vi "AssertLessThan_Tests.vi"(11 "error in":errorcluster) -> (15 "error out":errorcluster)   [LabVIEW 2016, in "DronaTest.lvlib"]
uses:
  DronaTest.lvlib
  APIs/Assert/AssertControlValue/LessOrEqual.vi
  <vilib>/addons/_JKI Toolkits/Caraya/classes/Assert/Assert Less Or Equal_Variant.vi
  APIs/Assert/AssertControlValue/Less.vi
  <vilib>/addons/_JKI Toolkits/Caraya/classes/Assert/Assert Less_Variant.vi
  <vilib>/addons/_JKI Toolkits/Caraya/classes/Assert/Assert Error.vi
  <vilib>/addons/_JKI Toolkits/Caraya/classes/Test/Test.lvclass
  Drona.lvlib
  <vilib>/addons/_JKI Toolkits/Caraya/classes/Assert/Assert.lvclass
  APIs/Assert/AssertControlValue/AssertControlValue.lvlib
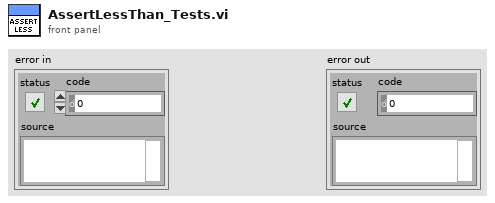
[diagram p1: front panel]
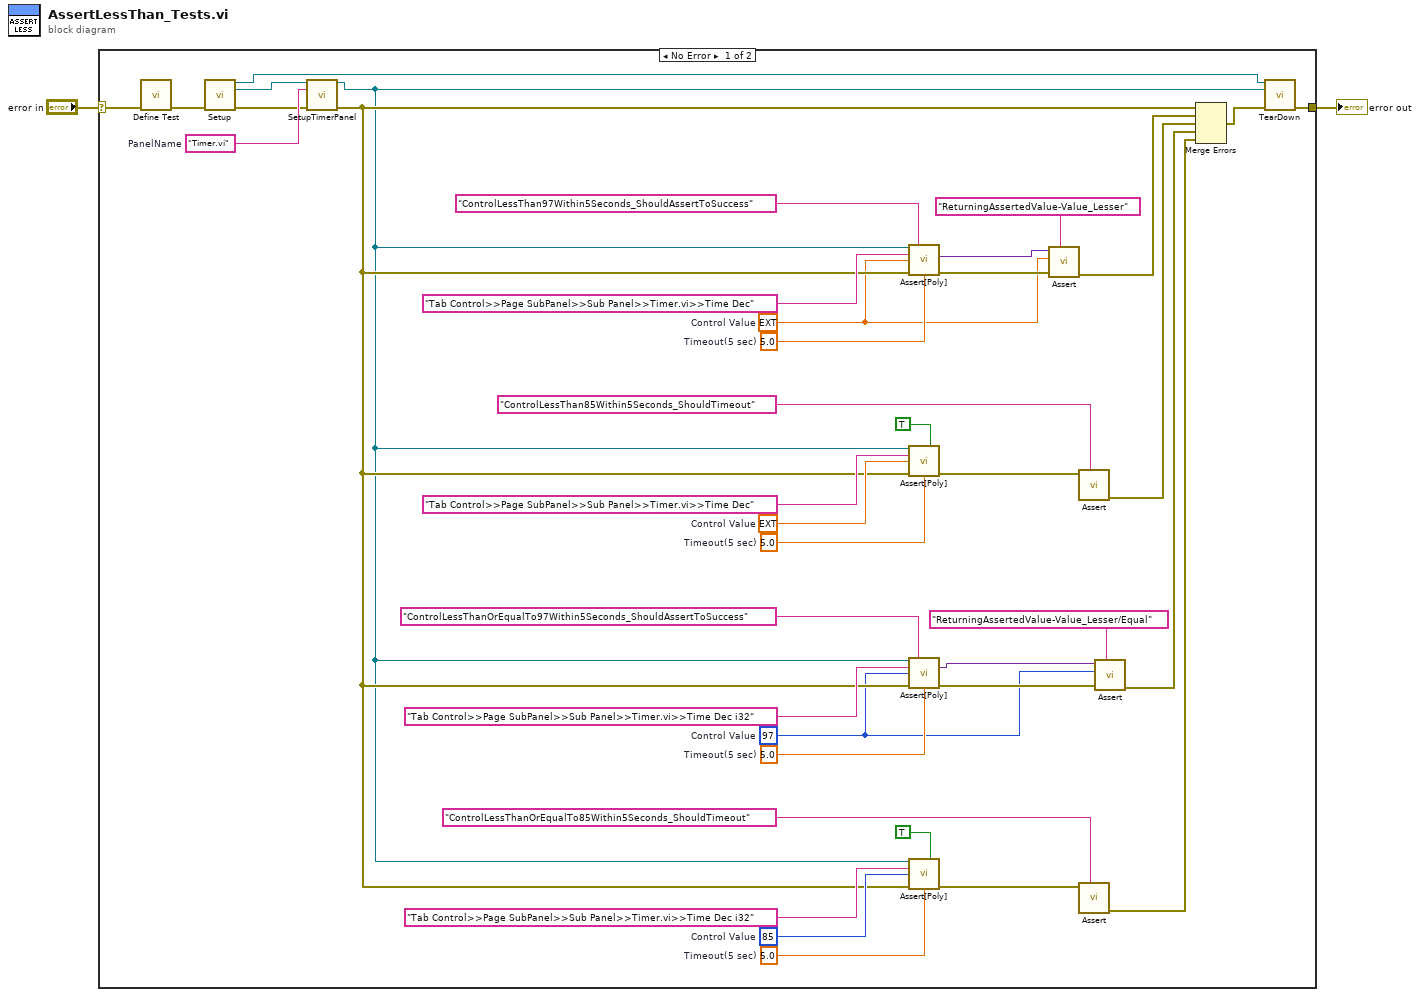
[diagram p0: block diagram]
diagram:
  n1 = case shown="No Error" "error in" {
    selector: "error in" -> [w42 w43]
    tunnel: [w17 w43] -> w1
    frame No Error {
      w21 = "Timer.vi"  # PanelName
      w35 = 5.0  # Timeout(5 sec)
      w3 = 97  # Control Value
      w36 = 5.0  # Timeout(5 sec)
      w37 = 85  # Control Value
      w30 = 5.0  # Timeout(5 sec)
      w9 = ext 97.0  # Control Value
      w29 = 5.0  # Timeout(5 sec)
      w28 = ext 85.0  # Control Value
      n2 = call <vilib>:"Define Test.vi"("error in (no error)"=w42) -> ("error out"=w16:errorcluster)  [unwired: 9 in, 1 out]
      n3 = call "Setup.vi"("error in (no error)"=w16) -> ("Application Ref"=w15:refnum<vi>, "VI out"=w19:refnum<vi>, "error out"=w20:errorcluster)  [unwired: 12 in]
      n4 = call "SetupTimerPanel.vi"("VI in"=w19, "Item Name"=w21, "error in (no error)"=w20) -> ("VI out"=w13:refnum<vi>, "error out"=w14:errorcluster)  [unwired: 11 in]
      n5 = call-poly "Assert[Poly].vi"("VI Reference In"=w13, "Test Label"="ControlLessThan97Within5Seconds_ShouldAssertToSuccess" ("string"), "Control Path"="Tab Control>>Page SubPanel>>Sub Panel>>Timer.vi>>Time Dec", "Control Value"=w9, "Error In"=w14, "Timeout(5 sec)"=w30) -> ("Asserted Value"=w10:variant, "Error Out"=w12:errorcluster)  [unwired: 7 in, 1 out]
      n6 = call-poly "Assert[Poly].vi"("VI Reference In"=w13, "Assert Only? (F)"=TRUE, "Control Path"="Tab Control>>Page SubPanel>>Sub Panel>>Timer.vi>>Time Dec", "Control Value"=w28, "Error In"=w14, "Timeout(5 sec)"=w29) -> ("Error Out"=w26:errorcluster)  [unwired: 7 in, 2 out]
      n7 = call-poly "Assert[Poly].vi"("VI Reference In"=w13, "Test Label"="ControlLessThanOrEqualTo97Within5Seconds_ShouldAssertToSuccess" ("string"), "Control Path"="Tab Control>>Page SubPanel>>Sub Panel>>Timer.vi>>Time Dec i32", "Control Value"=w3, "Error In"=w14, "Timeout(5 sec)"=w35) -> ("Asserted Value"=w4:variant, "Error Out"=w7:errorcluster)  [unwired: 7 in, 1 out]
      n8 = call-poly "Assert[Poly].vi"("VI Reference In"=w13, "Assert Only? (F)"=TRUE, "Control Path"="Tab Control>>Page SubPanel>>Sub Panel>>Timer.vi>>Time Dec i32", "Control Value"=w37, "Error In"=w14, "Timeout(5 sec)"=w36) -> ("Error Out"=w39:errorcluster)  [unwired: 7 in, 2 out]
      n9 = call-poly <vilib>:"Assert.vi"("Label"="ReturningAssertedValue-Value_Lesser", "error in (no error)"=w12, "Y"=w9, "X"=w10) -> ("error out"=w11:errorcluster)  [unwired: 6 in, 1 out]
      n10 = call-poly <vilib>:"Assert.vi"("Label"="ControlLessThan85Within5Seconds_ShouldTimeout" ("string"), "Error?"=w26) -> ("error out"=w23:errorcluster)  [unwired: 8 in, 1 out]
      n11 = call-poly <vilib>:"Assert.vi"("Label"="ControlLessThanOrEqualTo85Within5Seconds_ShouldTimeout" ("string"), "Error?"=w39) -> ("error out"=w22:errorcluster)  [unwired: 8 in, 1 out]
      n12 = call-poly <vilib>:"Assert.vi"("Label"="ReturningAssertedValue-Value_Lesser/Equal", "error in (no error)"=w7, "Y"=w3, "X"=w4) -> ("error out"=w6:errorcluster)  [unwired: 6 in, 1 out]
      n13 = Merge Errors(w14, w11, w23, w6, w22) -> (w18:errorcluster)
      n14 = call "TearDown.vi"("Application Ref"=w15, "VI in"=w13, "error in (no error)"=w18) -> ("error out"=w17:errorcluster)  [unwired: 12 in]
    }
    frame Error {
    }
  }
  "error out" <- w1
